vi "获取扫描电压.vi"(11 "数据":T1[](array[typedef])) -> (2 "负":dbl[](array[numeric]), 3 "正":dbl[](array[numeric]))   [LabVIEW 2020]
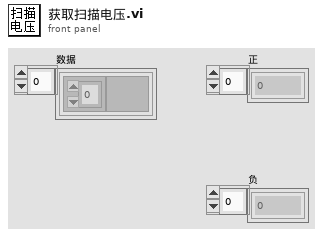
[diagram p1: front panel]
types:
  T1 = typedef "数据显示.xctl/波形数据定义.ctl" = cluster{"波形":dbl[][], "属性":variant}
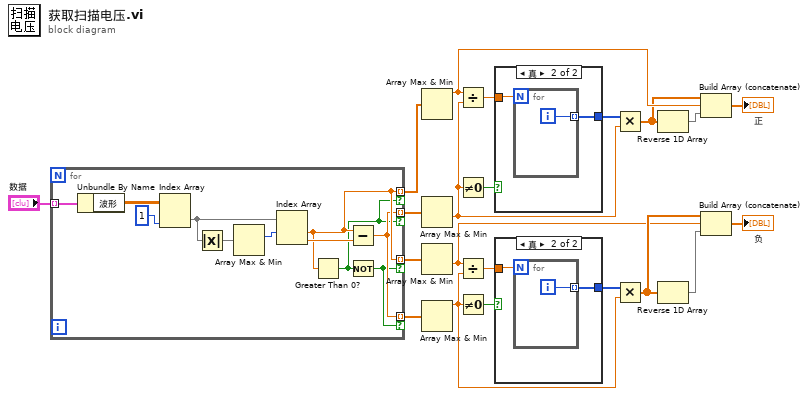
[diagram p0: block diagram]
diagram:
  n1 = for {
    tunnel: "数据" -> [w32] mode=indexing
    tunnel: [w25] -> w15 mode=indexing if=w23
    tunnel: [w24] -> w16 mode=indexing if=w23
    tunnel: [w25] -> w17 mode=indexing if=w22
    tunnel: [w24] -> w18 mode=indexing if=w22
    n2 = Unbundle By Name(w32) -> ("波形"=w29:dbl[][])
    n3 = Index Array(array=w29, index (col)=1 ("禁用的索引 (列)")) -> (element=w28:dbl[])  [unwired: 1 in]
    n4 = Absolute Value(x=w28) -> (abs(x)=w31:dbl[])
    n5 = Array Max & Min(array=w31) -> (max index (indices)=w30:i32)  [unwired: 3 out]
    n6 = Index Array(array=w28, index #1=w30) -> (element #1=w25:dbl, element #2=w26:dbl)  [unwired: 1 in]
    n7 = Greater Than 0?(x=w25) -> (x > 0?=w23:bool)
    n8 = Subtract(x=w25, y=w26) -> (x-y=w24:dbl)
    n9 = Not(x=w23) -> (.not. x?=w22:bool)
  }
  n10 = Array Max & Min(array=w15) -> (max value=w14:dbl)  [unwired: 3 out]
  n11 = Array Max & Min(array=w16) -> (min value=w3:dbl)  [unwired: 3 out]
  n12 = Array Max & Min(array=w17) -> (min value=w1:dbl)  [unwired: 3 out]
  n13 = Array Max & Min(array=w18) -> (max value=w5:dbl)  [unwired: 3 out]
  n14 = Divide(x=w14, y=w3) -> (x/y=w8:dbl)
  n15 = Not Equal To 0?(x=w3) -> (x != 0?=w2:bool)
  n16 = Divide(x=w1, y=w5) -> (x/y=w9:dbl)
  n17 = Not Equal To 0?(x=w5) -> (x != 0?=w4:bool)
  n18 = case shown="真" w2 {
    tunnel: w8 -> [_ w34]
    tunnel: [_ w33] -> w6
    frame False {
    }
    frame True {
      n19 = for {
        N: w34 -> [_]
        tunnel: [w35] -> w33 mode=indexing
        i -> [w35]
      }
    }
  }
  n20 = case shown="真" w4 {
    tunnel: w9 -> [_ w37]
    tunnel: [_ w36] -> w7
    frame False {
    }
    frame True {
      n21 = for {
        N: w37 -> [_]
        tunnel: [w38] -> w36 mode=indexing
        i -> [w38]
      }
    }
  }
  n22 = Multiply(x=w6, y=w3) -> (x*y=w13:dbl[])
  n23 = Multiply(x=w7, y=w5) -> (x*y=w10:dbl[])
  n24 = Reverse 1D Array(array=w13) -> (reversed array=w12:dbl[])
  n25 = Reverse 1D Array(array=w10) -> (reversed array=w11:dbl[])
  n26 = Build Array (concatenate)(w13, w14, w12) -> (→"正":dbl[])
  n27 = Build Array (concatenate)(w10, w1, w11) -> (→"负":dbl[])
